vi "Test RoundTrip Path.vi"(8 "error in (no error)":errorcluster) -> (0 "error out":errorcluster)   [LabVIEW 2013]
uses:
  <vilib>/addons/_JKI Toolkits/Caraya/classes/Test/Test.lvclass
  <vilib>/addons/_JKI Toolkits/Caraya/classes/Assert/Assert.lvclass
  src/JKI JSON Serialization.lvlib
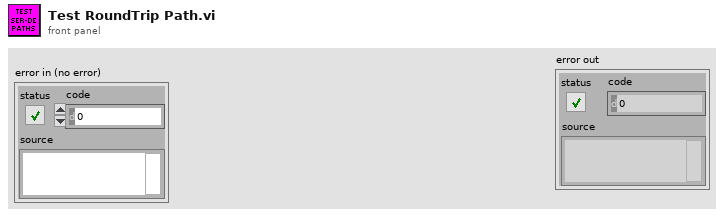
[diagram p1: front panel]
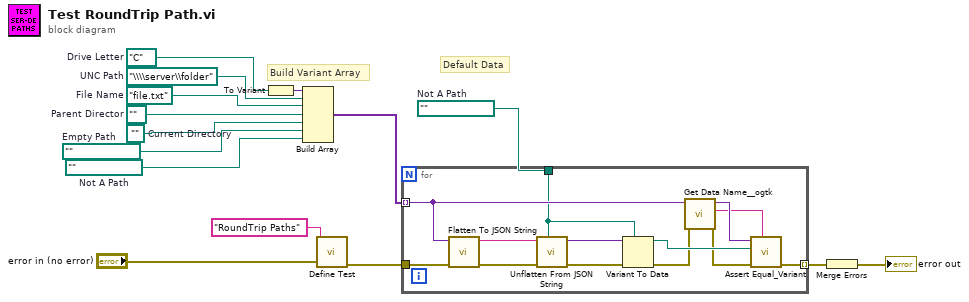
[diagram p0: block diagram]
diagram:
  w1 = path ""  # Not A Path
  w5 = path ""  # Not A Path
  w10 = path "file.txt"  # File Name
  w11 = path "\\\\server\\folder"  # UNC Path
  w4 = path "C:/"  # Drive Letter
  w7 = path ""  # Empty Path
  w8 = path ""  # Current Directory
  w9 = path ".."  # Parent Director
  # "Build Variant Array"
  # "Default Data"
  n1 = To Variant(anything=w4) -> (Variant=w2:variant)
  n2 = Build Array(w2, w11, w10, w9, w8, w7, w5) -> (w3:variant[])
  n3 = call <vilib>:"Define Test.vi"("error in (no error)"="error in (no error)", "Label (VI Title)"="RoundTrip Paths") -> ("error out"=w6:errorcluster)  [unwired: 9 in]
  n4 = for {
    tunnel: w3 -> [w24] mode=indexing
    tunnel: w6 -> [w19]
    tunnel: [w18] -> w13 mode=indexing
    tunnel: w1 -> [w17]
    n5 = call "Flatten To JSON String.vi"("error in (no error)"=w19, "Variant"=w24) -> ("error out"=w28:errorcluster, "JSON String"=w16:string)  [unwired: 8 in]
    n6 = call "Unflatten From JSON String.vi"("Type and Defaults"=w17, "error in (no error)"=w28, "JSON String"=w16) -> ("error out"=w25:errorcluster, "Variant"=w27:variant)  [unwired: 7 in]
    n7 = Variant To Data(error in=w25, type=w17, Variant=w27) -> (data=w26:path, error out=w21:errorcluster)
    n8 = call <userlib>:"Get Data Name__ogtk.vi"("error in (no error)"=w21, "Data"=w24) -> ("error out"=w20:errorcluster, "Data Name"=w22:string, "Data dup"=w23:variant)  [unwired: 7 in]
    n9 = call <vilib>:"Assert Equal_Variant.vi"("Label"=w22, "error in (no error)"=w20, "Y"=w26, "X"=w23) -> ("error out"=w18:errorcluster)  [unwired: 7 in]
  }
  n10 = Merge Errors(w13) -> (→"error out":errorcluster)
